vi "RemoteVI Complex Fixture Arrange.vi"(0 "Fixture":path, 1 "Views":path[](array[path]), 11 "error in":errorcluster) -> (4 "problems":string[](array[string]), 15 "error out":errorcluster)   [LabVIEW 2020]
doc: "Build tool of RemoteVI Complex Fixture.vi: run it after RemoteVI Complex Fixture Paste.vi, with the fixture idle; it can be run again (every step sets, nothing is added). Lays the panel out: each control is moved (GObject Move) into its pane (0 left, 1 toolbar, 2 main) or into a page of the tab control Settings and placed at fixed panel-area coordinates (the pane coordinates are the wanted point minus where the pane's 0,0 lands: CvtPaneToPanelCoords, CvtPanelToScreenCoords, minus Panel Bounds - placing relative to the pane's Position drifted from run to run) or relative to Settings. The toolbar holds Inspector, View, Stop and Status, the left pane Nav, Results and Steps (taller than the pane, so it scrolls) and the hidden Log Path and error out, the main pane Settings; page Acquisition holds Channel, Rate, Level and Data File, page Display holds Scope, page Viewer (added with Add Page when the tab has two) the subpanel Viewer. Then: pages named Acquisition, Display and Viewer with fixed 110 px tabs, Stop and Inspector switch when released, Data File with its browse button, Results with column headers and three rows, Steps three elements high, tip strips on Rate, on Gain inside Channel and on Nav, the main pane scaling Settings with the pane (Pane Set Scaling, Scale Single Object), the left pane's vertical scrollbar always on, the window 1180 x 760; in View A, View B and the inspector (Views) the Quit switches hidden and tip strips set. Saves the fixture and the views. problems lists every row or step that returned an error, with its code; the run goes on."
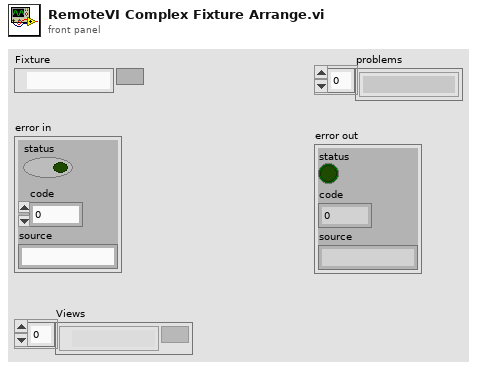
[diagram p1: front panel]
types:
  T1 = enum16{"Always On", "Always Off", "Off While Running"}
  T2 = enum16{"No Scaling", "Scale All Objects", "Scale Single Object"}
  T3 = cluster{"Left":i32, "Top":i32, "Right":i32, "Bottom":i32}
  T4 = typedef "LVRectTypeDef.ctl" = cluster{"left":i16, "top":i16, "right":i16, "bottom":i16}
  T5 = typedef "LVPositionTypeDef.ctl" = cluster{"Left":i32, "Top":i32}
  T6 = typedef "LVPointTypeDef.ctl" = cluster{"Horizontal":i16, "Vertical":i16}
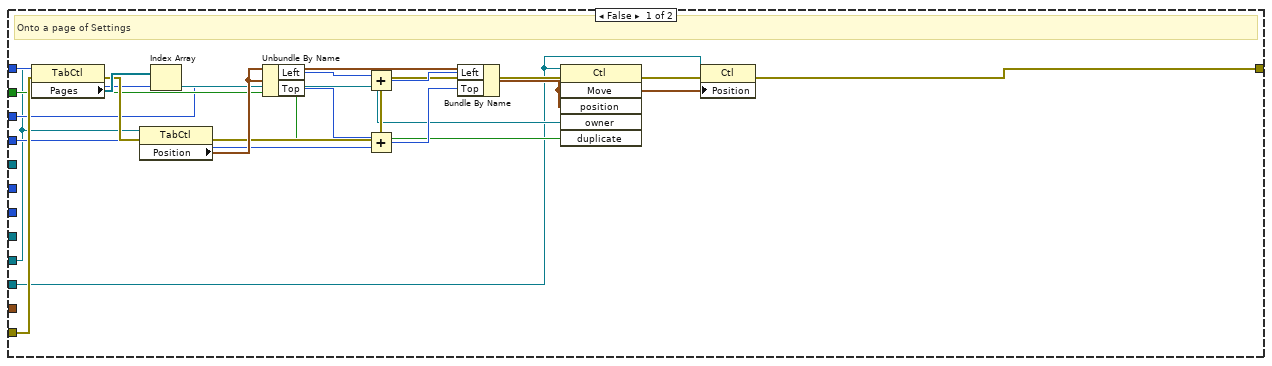
[diagram p2: hidden frame]
diagram:
  w221 = FALSE  # hidden
  w220 = string[] ["Apply view A", "Run view B", "Apply the note"]  # tips
  w219 = string[] ["A Apply", "B Run", "Apply"]  # tip labels
  w218 = string[] ["A Quit", "B Quit", "Inspector Quit"]  # quit labels
  w215 = "VertScrollbarVisibility %d"  # fmt
  w212 = T1."Always On"  # always on
  w209 = "Set Scaling %d"  # fmt
  w206 = T2."Scale Single Object"  # scale single object
  w204 = 2  # two
  w202 = "Status Label.Visible %d"  # fmt
  w198 = FALSE  # value
  w194 = string[] ["Status"]  # Status
  w192 = "View Label.Visible %d"  # fmt
  w188 = FALSE  # value
  w184 = string[] ["View"]  # View
  w182 = "Nav TipStrip %d"  # fmt
  w178 = "Pick a section"  # value
  w174 = string[] ["Nav"]  # Nav
  w172 = "Gain TipStrip %d"  # fmt
  w168 = "Channel gain"  # value
  w164 = string[] ["Gain"]  # Gain
  w162 = "Rate TipStrip %d"  # fmt
  w158 = "Sample rate"  # value
  w154 = string[] ["Rate"]  # Rate
  w152 = "Steps Number of Rows %d"  # fmt
  w148 = u32 3  # value
  w145 = refnum<vi> refnum  # class
  w141 = string[] ["Steps"]  # Steps
  w139 = "Results Value %d"  # fmt
  w135 = string[][] [["Init", "1"], ["Run", "2"], ["Stop", "3"]]  # value
  w132 = refnum<vi> refnum  # class
  w128 = string[] ["Results"]  # Results
  w126 = "Results Column Header Strings[] %d"  # fmt
  w122 = string[] ["Step", "Value"]  # value
  w119 = refnum<vi> refnum  # class
  w115 = string[] ["Results"]  # Results
  w113 = "Results Visible Items:Column Headers Visible %d"  # fmt
  w109 = TRUE  # value
  w106 = refnum<vi> refnum  # class
  w102 = string[] ["Results"]  # Results
  w100 = "Data File Browse Button:Visible %d"  # fmt
  w96 = TRUE  # value
  w93 = refnum<vi> refnum  # class
  w89 = string[] ["Data File"]  # Data File
  w87 = "error out Visible %d"  # fmt
  w83 = FALSE  # value
  w79 = string[] ["error out"]  # error out
  w77 = "Log Path Visible %d"  # fmt
  w73 = FALSE  # value
  w69 = string[] ["Log Path"]  # Log Path
  w67 = "Inspector Mechanical Action %d"  # fmt
  w63 = u32 1  # value
  w60 = refnum<vi> refnum  # class
  w56 = string[] ["Inspector"]  # Inspector
  w54 = "Stop Mechanical Action %d"  # fmt
  w50 = u32 1  # value
  w47 = refnum<vi> refnum  # class
  w43 = string[] ["Stop"]  # Stop
  w36 = FALSE  # no duplicate
  w35 = cluster{"Left":i32, "Top":i32}[] [{"Left"=300, "Top"=6}, {"Left"=420, "Top"=7}, {"Left"=14, "Top"=28}, {"Left"=120, "Top"=28}, {"Left"=14, "Top"=84}, {"Left"=14, "Top"=310}, {"Left"=14, "Top"=600}, {"Left"=14, "Top"=860}, {"Left"=14, "Top"=900}, {"Left"=300, "Top"=52}, {"Left"=20, "Top"=50}, {"Left"=230, "Top"=40}, {"Left"=390, "Top"=40}, {"Left"=20, "Top"=220}, {"Left"=10, "Top"=40}, {"Left"=20, "Top"=50}]  # offsets
  w34 = i32[] [-1, -1, -1, -1, -1, -1, -1, -1, -1, -1, 0, 0, 0, 0, 1, 2]  # pages
  w33 = i32[] [1, 1, 0, 0, 0, 0, 0, 0, 0, 2, 2, 2, 2, 2, 2, 2]  # panes
  w32 = string[] ["View", "Status", "Inspector", "Stop", "Nav", "Results", "Steps", "Log Path", "error out", "Settings", "Channel", "Rate", "Level", "Data File", "Scope", "Viewer"]  # labels
  w29 = string[] ["Acquisition", "Display", "Viewer"]  # page names
  w25 = 3  # three
  w21 = cluster{"Width":i32, "Height":i32} {"Width"=110, "Height"=23}  # tab dimension
  w20 = 2  # fixed tab size
  w17 = refnum<vi> refnum  # tab class
  w15 = 1  # one
  w14 = 0  # zero
  w11 = string[] ["Settings", "Gain"]  # settings
  w9 = T3 {"Left"=80, "Top"=80, "Right"=1260, "Bottom"=840}  # window
  # "Lay the panel out, then save"
  n1 = for {
    tunnel: "Views" -> [w229] mode=indexing
    tunnel: w218 -> [w230] mode=indexing
    tunnel: w219 -> [w231] mode=indexing
    tunnel: w220 -> [w232] mode=indexing
    tunnel: w221 -> [w233]
    tunnel: w14 -> [w234]
    tunnel: w15 -> [w235]
    tunnel: [w251] -> w222 mode=indexing
    w250 = "view %s %d"  # fmt
    # "Each view"
    n2 = Open VI Reference(vi path=w229) -> (vi reference=w236:refnum<vi>, error out=w237:errorcluster)  [unwired: 5 in]
    n3 = Build Array(w230, w231) -> (w240:string[])
    n4 = property class="VI"(reference=w236, error in=w237) -> (error out=w238:errorcluster, "Front Panel"=w239:refnum<vi>)  [unwired: 1 out]
    n5 = call "RemoteVI Complex Fixture Find Controls.vi"("Panel"=w239, "labels"=w240, "error in"=w238) -> ("Controls"=w241:refnum<vi>[], "error out"=w242:errorcluster)  [unwired: 11 in]
    n6 = Index Array(array=w241, index=w234) -> (element=w243:refnum<vi>)
    n7 = Index Array(array=w241, index=w235) -> (element=w244:refnum<vi>)
    n8 = property class="Ctl"(reference=w243, error in=w242, "Visible"=w233) -> (error out=w245:errorcluster)  [unwired: 1 out]
    n9 = property class="Ctl"(reference=w244, error in=w245, "TipStrip"=w232) -> (error out=w246:errorcluster)  [unwired: 1 out]
    n10 = invoke class="VI" method="Save.Instrument"(reference=w236, error in=w246) -> (error out=w247:errorcluster)  [unwired: 4 in, 5 out]
    n11 = Close Reference(reference=w236, error in (no error)=w247) -> (error out=w248:errorcluster)
    n12 = Unbundle By Name(w248) -> ("code"=w249:i32)
    n13 = Format Into String(format string=w250, w230, w249) -> (resulting string=w251:string)  [unwired: 2 in, 1 out]
  }
  n14 = Open VI Reference(vi path="Fixture", error in (no error)="error in") -> (vi reference=w3:refnum<vi>, error out=w4:errorcluster)  [unwired: 4 in]
  n15 = property class="VI"(reference=w3) -> ("Front Panel Window:Panel Bounds"=w37:T4)  [unwired: 1 in, 2 out]
  n16 = property class="VI"(reference=w3, error in=w4) -> (error out=w5:errorcluster, "Front Panel"=w6:refnum<vi>)  [unwired: 1 out]
  n17 = property class="Pnl"(reference=w6, error in=w5) -> (error out=w7:errorcluster, "Panes[]"=w8:refnum<vi>[])  [unwired: 1 out]
  n18 = Unbundle By Name(w37) -> ("left"=w38:i16, "top"=w39:i16)
  n19 = property class="VI"(reference=w3, error in=w7, "Front Panel Window:Panel Bounds"=w9) -> (error out=w10:errorcluster)  [unwired: 1 out]
  n20 = Index Array(array=w8, index=w204) -> (element=w205:refnum<vi>)
  n21 = Index Array(array=w8, index=w14) -> (element=w211:refnum<vi>)
  n22 = call "RemoteVI Complex Fixture Find Controls.vi"("Panel"=w6, "labels"=w11, "error in"=w10) -> ("Controls"=w12:refnum<vi>[], "error out"=w13:errorcluster)  [unwired: 11 in]
  n23 = Index Array(array=w12, index=w14) -> (element=w16:refnum<vi>)
  n24 = To More Specific Class(target class=w17, reference=w16, error in=w13) -> (specific class reference=w18:refnum<vi>, error out=w19:errorcluster)
  n25 = property class="TabCtl"(reference=w18, error in=w19, "Tab Size"=w20, "Fixed Tab Dimension"=w21) -> (error out=w22:errorcluster, "Pages"=w23:refnum<vi>[])  [unwired: 1 out]
  n26 = Array Size(array=w23) -> (size(s)=w24:i32)
  n27 = Less?(x=w24, y=w25) -> (x < y?=w26:bool)
  n28 = case shown="True" w26 {
    tunnel: w18 -> [_ w254]
    tunnel: w22 -> [w252 w255]
    tunnel: w23 -> [w253 _]
    tunnel: [w253 w260] -> w27
    tunnel: [w252 w259] -> w28
    frame False {
    }
    frame True {
      w257 = TRUE  # after
      w256 = 1  # after page 1
      # "Two pages: add the third (Viewer)"
      n29 = invoke class="TabCtl" method="Add Page"(reference=w254, error in=w255, "Page"=w256, "After"=w257) -> (error out=w258:errorcluster)  [unwired: 1 in, 4 out]
      n30 = property class="TabCtl"(reference=w254, error in=w258) -> (error out=w259:errorcluster, "Pages"=w260:refnum<vi>[])  [unwired: 1 out]
    }
  }
  n31 = for {
    tunnel: w29 -> [w262] mode=indexing
    tunnel: w27 -> [w261] mode=indexing
    shift-right: [w264] -> w30
    shift-left: w28 -> [w263]
    # "Name the pages"
    n32 = property class="Page"(reference=w261, error in=w263, "Page Label"=w262, "TabCaption"=w262) -> (error out=w264:errorcluster)  [unwired: 1 out]
  }
  n33 = call <vilib>:"Clear Errors.vi"("error in (no error)"=w30) -> ("error out"=w31:errorcluster)  [unwired: 5 in, 1 out]
  n34 = for {
    tunnel: w32 -> [w265] mode=indexing
    tunnel: w33 -> [w266] mode=indexing
    tunnel: w34 -> [w267] mode=indexing
    tunnel: w35 -> [w268] mode=indexing
    tunnel: w36 -> [w272]
    tunnel: w6 -> [w269]
    tunnel: w8 -> [w270]
    tunnel: w38 -> [w274]
    tunnel: w39 -> [w275]
    tunnel: w18 -> [w271]
    tunnel: w31 -> [w273]
    tunnel: [w287] -> w41
    tunnel: [w290] -> w40 mode=indexing
    w289 = "%s %d"  # fmt
    w279 = 0  # zero
    # "Move each control into its pane or page and place it"
    n35 = Build Array(w265) -> (w276:string[])
    n36 = Less Than 0?(x=w267) -> (x < 0?=w284:bool)
    n37 = Unbundle By Name(w268) -> ("Left"=w285:i32, "Top"=w286:i32)
    n38 = Index Array(array=w270, index=w266) -> (element=w281:refnum<vi>)
    n39 = call "RemoteVI Complex Fixture Find Controls.vi"("Panel"=w269, "labels"=w276, "error in"=w273) -> ("Controls"=w277:refnum<vi>[], "error out"=w278:errorcluster)  [unwired: 11 in]
    n40 = property class="Pane"(reference=w281, error in=w278) -> (error out=w282:errorcluster, "Position"=w283:T5)  [unwired: 1 out]
    n41 = Index Array(array=w277, index=w279) -> (element=w280:refnum<vi>)
    n42 = case shown="True" w284 {
      tunnel: w267 -> [w293 _]
      tunnel: w272 -> [w296 w314]
      tunnel: w285 -> [w294 w312]
      tunnel: w286 -> [w295 w313]
      tunnel: w269 -> [_ w316]
      tunnel: w274 -> [_ w317]
      tunnel: w275 -> [_ w318]
      tunnel: w281 -> [_ w311]
      tunnel: w271 -> [w292 _]
      tunnel: w280 -> [w291 w310]
      tunnel: w283 -> [_ _]
      tunnel: w282 -> [w297 w315]
      tunnel: [w309 w333] -> w287
      frame False {
        # "Onto a page of Settings"
        n43 = property class="TabCtl"(reference=w292, error in=w297) -> (error out=w298:errorcluster, "Pages"=w299:refnum<vi>[])  [unwired: 1 out]
        n44 = property class="TabCtl"(reference=w292, error in=w298) -> (error out=w301:errorcluster, "Position"=w302:T5)  [unwired: 1 out]
        n45 = Index Array(array=w299, index=w293) -> (element=w300:refnum<vi>)
        n46 = Unbundle By Name(w302) -> ("Left"=w303:i32, "Top"=w304:i32)
        n47 = Add(x=w303, y=w294) -> (x+y=w305:i32)
        n48 = Add(x=w304, y=w295) -> (x+y=w306:i32)
        n49 = Bundle By Name(cluster=w302, "Left"=w305, "Top"=w306) -> (w307:T5)
        n50 = invoke class="Ctl" method="Move"(reference=w291, error in=w301, "position"=w307, "owner"=w300, "duplicate"=w296) -> (error out=w308:errorcluster)  [unwired: 1 in, 5 out]
        n51 = property class="Ctl"(reference=w291, error in=w308, "Position"=w307) -> (error out=w309:errorcluster)  [unwired: 1 out]
      }
      frame True {
        w330 = cluster{"Left":i32, "Top":i32} {"Left"=0, "Top"=0}  # position
        w319 = cluster{"Horizontal":i32, "Vertical":i32} {"Horizontal"=0, "Vertical"=0}  # pane origin
        # "Into the pane"
        n52 = invoke class="Pane" method="CvtPaneToPanelCoords"(reference=w311, error in=w315, "PaneCoords"=w319) -> (error out=w320:errorcluster, "PanelCoords"=w321:T6)  [unwired: 2 in, 3 out]
        n53 = invoke class="Pnl" method="CvtPanelToScreenCoords"(reference=w316, error in=w320, "PanelCoords"=w321) -> (error out=w322:errorcluster, "ScreenCoords"=w323:T6)  [unwired: 2 in, 3 out]
        n54 = Unbundle By Name(w323) -> ("Horizontal"=w324:i16, "Vertical"=w325:i16)
        n55 = Subtract(x=w324, y=w317) -> (x-y=w326:i16)
        n56 = Subtract(x=w325, y=w318) -> (x-y=w327:i16)
        n57 = Subtract(x=w312, y=w326) -> (x-y=w328:i32)
        n58 = Subtract(x=w313, y=w327) -> (x-y=w329:i32)
        n59 = Bundle By Name(cluster=w330, "Left"=w328, "Top"=w329) -> (w331:cluster{"Left":i32, "Top":i32})
        n60 = invoke class="Ctl" method="Move"(reference=w310, error in=w322, "position"=w331, "owner"=w311, "duplicate"=w314) -> (error out=w332:errorcluster)  [unwired: 1 in, 5 out]
        n61 = property class="Ctl"(reference=w310, error in=w332, "Position"=w331) -> (error out=w333:errorcluster)  [unwired: 1 out]
      }
    }
    n62 = Unbundle By Name(w287) -> ("code"=w288:i32)
    n63 = Format Into String(format string=w289, w265, w288) -> (resulting string=w290:string)  [unwired: 2 in, 1 out]
  }
  n64 = call <vilib>:"Clear Errors.vi"("error in (no error)"=w41) -> ("error out"=w42:errorcluster)  [unwired: 5 in, 1 out]
  n65 = call "RemoteVI Complex Fixture Find Controls.vi"("Panel"=w6, "labels"=w43, "error in"=w42) -> ("Controls"=w44:refnum<vi>[], "error out"=w45:errorcluster)  [unwired: 11 in]
  n66 = Index Array(array=w44, index=w14) -> (element=w46:refnum<vi>)
  n67 = To More Specific Class(target class=w47, reference=w46, error in=w45) -> (specific class reference=w48:refnum<vi>, error out=w49:errorcluster)
  n68 = property class="Bool"(reference=w48, error in=w49, "Mechanical Action"=w50) -> (error out=w51:errorcluster)  [unwired: 1 out]
  n69 = Unbundle By Name(w51) -> ("code"=w52:i32)
  n70 = call <vilib>:"Clear Errors.vi"("error in (no error)"=w51) -> ("error out"=w53:errorcluster)  [unwired: 5 in, 1 out]
  n71 = Format Into String(format string=w54, w52) -> (resulting string=w55:string)  [unwired: 2 in, 1 out]
  n72 = call "RemoteVI Complex Fixture Find Controls.vi"("Panel"=w6, "labels"=w56, "error in"=w53) -> ("Controls"=w57:refnum<vi>[], "error out"=w58:errorcluster)  [unwired: 11 in]
  n73 = Index Array(array=w57, index=w14) -> (element=w59:refnum<vi>)
  n74 = To More Specific Class(target class=w60, reference=w59, error in=w58) -> (specific class reference=w61:refnum<vi>, error out=w62:errorcluster)
  n75 = property class="Bool"(reference=w61, error in=w62, "Mechanical Action"=w63) -> (error out=w64:errorcluster)  [unwired: 1 out]
  n76 = Unbundle By Name(w64) -> ("code"=w65:i32)
  n77 = call <vilib>:"Clear Errors.vi"("error in (no error)"=w64) -> ("error out"=w66:errorcluster)  [unwired: 5 in, 1 out]
  n78 = Format Into String(format string=w67, w65) -> (resulting string=w68:string)  [unwired: 2 in, 1 out]
  n79 = call "RemoteVI Complex Fixture Find Controls.vi"("Panel"=w6, "labels"=w69, "error in"=w66) -> ("Controls"=w70:refnum<vi>[], "error out"=w71:errorcluster)  [unwired: 11 in]
  n80 = Index Array(array=w70, index=w14) -> (element=w72:refnum<vi>)
  n81 = property class="Ctl"(reference=w72, error in=w71, "Visible"=w73) -> (error out=w74:errorcluster)  [unwired: 1 out]
  n82 = Unbundle By Name(w74) -> ("code"=w75:i32)
  n83 = call <vilib>:"Clear Errors.vi"("error in (no error)"=w74) -> ("error out"=w76:errorcluster)  [unwired: 5 in, 1 out]
  n84 = Format Into String(format string=w77, w75) -> (resulting string=w78:string)  [unwired: 2 in, 1 out]
  n85 = call "RemoteVI Complex Fixture Find Controls.vi"("Panel"=w6, "labels"=w79, "error in"=w76) -> ("Controls"=w80:refnum<vi>[], "error out"=w81:errorcluster)  [unwired: 11 in]
  n86 = Index Array(array=w80, index=w14) -> (element=w82:refnum<vi>)
  n87 = property class="Ctl"(reference=w82, error in=w81, "Visible"=w83) -> (error out=w84:errorcluster)  [unwired: 1 out]
  n88 = Unbundle By Name(w84) -> ("code"=w85:i32)
  n89 = call <vilib>:"Clear Errors.vi"("error in (no error)"=w84) -> ("error out"=w86:errorcluster)  [unwired: 5 in, 1 out]
  n90 = Format Into String(format string=w87, w85) -> (resulting string=w88:string)  [unwired: 2 in, 1 out]
  n91 = call "RemoteVI Complex Fixture Find Controls.vi"("Panel"=w6, "labels"=w89, "error in"=w86) -> ("Controls"=w90:refnum<vi>[], "error out"=w91:errorcluster)  [unwired: 11 in]
  n92 = Index Array(array=w90, index=w14) -> (element=w92:refnum<vi>)
  n93 = To More Specific Class(target class=w93, reference=w92, error in=w91) -> (specific class reference=w94:refnum<vi>, error out=w95:errorcluster)
  n94 = property class="Path"(reference=w94, error in=w95, "Browse Button:Visible"=w96) -> (error out=w97:errorcluster)  [unwired: 1 out]
  n95 = Unbundle By Name(w97) -> ("code"=w98:i32)
  n96 = call <vilib>:"Clear Errors.vi"("error in (no error)"=w97) -> ("error out"=w99:errorcluster)  [unwired: 5 in, 1 out]
  n97 = Format Into String(format string=w100, w98) -> (resulting string=w101:string)  [unwired: 2 in, 1 out]
  n98 = call "RemoteVI Complex Fixture Find Controls.vi"("Panel"=w6, "labels"=w102, "error in"=w99) -> ("Controls"=w103:refnum<vi>[], "error out"=w104:errorcluster)  [unwired: 11 in]
  n99 = Index Array(array=w103, index=w14) -> (element=w105:refnum<vi>)
  n100 = To More Specific Class(target class=w106, reference=w105, error in=w104) -> (specific class reference=w107:refnum<vi>, error out=w108:errorcluster)
  n101 = property class="Tbl"(reference=w107, error in=w108, "Visible Items:Column Headers Visible"=w109) -> (error out=w110:errorcluster)  [unwired: 1 out]
  n102 = Unbundle By Name(w110) -> ("code"=w111:i32)
  n103 = call <vilib>:"Clear Errors.vi"("error in (no error)"=w110) -> ("error out"=w112:errorcluster)  [unwired: 5 in, 1 out]
  n104 = Format Into String(format string=w113, w111) -> (resulting string=w114:string)  [unwired: 2 in, 1 out]
  n105 = call "RemoteVI Complex Fixture Find Controls.vi"("Panel"=w6, "labels"=w115, "error in"=w112) -> ("Controls"=w116:refnum<vi>[], "error out"=w117:errorcluster)  [unwired: 11 in]
  n106 = Index Array(array=w116, index=w14) -> (element=w118:refnum<vi>)
  n107 = To More Specific Class(target class=w119, reference=w118, error in=w117) -> (specific class reference=w120:refnum<vi>, error out=w121:errorcluster)
  n108 = property class="Tbl"(reference=w120, error in=w121, "Column Header Strings[]"=w122) -> (error out=w123:errorcluster)  [unwired: 1 out]
  n109 = Unbundle By Name(w123) -> ("code"=w124:i32)
  n110 = call <vilib>:"Clear Errors.vi"("error in (no error)"=w123) -> ("error out"=w125:errorcluster)  [unwired: 5 in, 1 out]
  n111 = Format Into String(format string=w126, w124) -> (resulting string=w127:string)  [unwired: 2 in, 1 out]
  n112 = call "RemoteVI Complex Fixture Find Controls.vi"("Panel"=w6, "labels"=w128, "error in"=w125) -> ("Controls"=w129:refnum<vi>[], "error out"=w130:errorcluster)  [unwired: 11 in]
  n113 = Index Array(array=w129, index=w14) -> (element=w131:refnum<vi>)
  n114 = To More Specific Class(target class=w132, reference=w131, error in=w130) -> (specific class reference=w133:refnum<vi>, error out=w134:errorcluster)
  n115 = property class="Tbl"(reference=w133, error in=w134, "Value"=w135) -> (error out=w136:errorcluster)  [unwired: 1 out]
  n116 = Unbundle By Name(w136) -> ("code"=w137:i32)
  n117 = call <vilib>:"Clear Errors.vi"("error in (no error)"=w136) -> ("error out"=w138:errorcluster)  [unwired: 5 in, 1 out]
  n118 = Format Into String(format string=w139, w137) -> (resulting string=w140:string)  [unwired: 2 in, 1 out]
  n119 = call "RemoteVI Complex Fixture Find Controls.vi"("Panel"=w6, "labels"=w141, "error in"=w138) -> ("Controls"=w142:refnum<vi>[], "error out"=w143:errorcluster)  [unwired: 11 in]
  n120 = Index Array(array=w142, index=w14) -> (element=w144:refnum<vi>)
  n121 = To More Specific Class(target class=w145, reference=w144, error in=w143) -> (specific class reference=w146:refnum<vi>, error out=w147:errorcluster)
  n122 = property class="Arr"(reference=w146, error in=w147, "Number of Rows"=w148) -> (error out=w149:errorcluster)  [unwired: 1 out]
  n123 = Unbundle By Name(w149) -> ("code"=w150:i32)
  n124 = call <vilib>:"Clear Errors.vi"("error in (no error)"=w149) -> ("error out"=w151:errorcluster)  [unwired: 5 in, 1 out]
  n125 = Format Into String(format string=w152, w150) -> (resulting string=w153:string)  [unwired: 2 in, 1 out]
  n126 = call "RemoteVI Complex Fixture Find Controls.vi"("Panel"=w6, "labels"=w154, "error in"=w151) -> ("Controls"=w155:refnum<vi>[], "error out"=w156:errorcluster)  [unwired: 11 in]
  n127 = Index Array(array=w155, index=w14) -> (element=w157:refnum<vi>)
  n128 = property class="Ctl"(reference=w157, error in=w156, "TipStrip"=w158) -> (error out=w159:errorcluster)  [unwired: 1 out]
  n129 = Unbundle By Name(w159) -> ("code"=w160:i32)
  n130 = call <vilib>:"Clear Errors.vi"("error in (no error)"=w159) -> ("error out"=w161:errorcluster)  [unwired: 5 in, 1 out]
  n131 = Format Into String(format string=w162, w160) -> (resulting string=w163:string)  [unwired: 2 in, 1 out]
  n132 = call "RemoteVI Complex Fixture Find Controls.vi"("Panel"=w6, "labels"=w164, "error in"=w161) -> ("Controls"=w165:refnum<vi>[], "error out"=w166:errorcluster)  [unwired: 11 in]
  n133 = Index Array(array=w165, index=w14) -> (element=w167:refnum<vi>)
  n134 = property class="Ctl"(reference=w167, error in=w166, "TipStrip"=w168) -> (error out=w169:errorcluster)  [unwired: 1 out]
  n135 = Unbundle By Name(w169) -> ("code"=w170:i32)
  n136 = call <vilib>:"Clear Errors.vi"("error in (no error)"=w169) -> ("error out"=w171:errorcluster)  [unwired: 5 in, 1 out]
  n137 = Format Into String(format string=w172, w170) -> (resulting string=w173:string)  [unwired: 2 in, 1 out]
  n138 = call "RemoteVI Complex Fixture Find Controls.vi"("Panel"=w6, "labels"=w174, "error in"=w171) -> ("Controls"=w175:refnum<vi>[], "error out"=w176:errorcluster)  [unwired: 11 in]
  n139 = Index Array(array=w175, index=w14) -> (element=w177:refnum<vi>)
  n140 = property class="Ctl"(reference=w177, error in=w176, "TipStrip"=w178) -> (error out=w179:errorcluster)  [unwired: 1 out]
  n141 = Unbundle By Name(w179) -> ("code"=w180:i32)
  n142 = call <vilib>:"Clear Errors.vi"("error in (no error)"=w179) -> ("error out"=w181:errorcluster)  [unwired: 5 in, 1 out]
  n143 = Format Into String(format string=w182, w180) -> (resulting string=w183:string)  [unwired: 2 in, 1 out]
  n144 = call "RemoteVI Complex Fixture Find Controls.vi"("Panel"=w6, "labels"=w184, "error in"=w181) -> ("Controls"=w185:refnum<vi>[], "error out"=w186:errorcluster)  [unwired: 11 in]
  n145 = Index Array(array=w185, index=w14) -> (element=w187:refnum<vi>)
  n146 = property class="Ctl"(reference=w187, error in=w186, "Label.Visible"=w188) -> (error out=w189:errorcluster)  [unwired: 1 out]
  n147 = Unbundle By Name(w189) -> ("code"=w190:i32)
  n148 = call <vilib>:"Clear Errors.vi"("error in (no error)"=w189) -> ("error out"=w191:errorcluster)  [unwired: 5 in, 1 out]
  n149 = Format Into String(format string=w192, w190) -> (resulting string=w193:string)  [unwired: 2 in, 1 out]
  n150 = call "RemoteVI Complex Fixture Find Controls.vi"("Panel"=w6, "labels"=w194, "error in"=w191) -> ("Controls"=w195:refnum<vi>[], "error out"=w196:errorcluster)  [unwired: 11 in]
  n151 = Index Array(array=w195, index=w14) -> (element=w197:refnum<vi>)
  n152 = property class="Ctl"(reference=w197, error in=w196, "Label.Visible"=w198) -> (error out=w199:errorcluster)  [unwired: 1 out]
  n153 = Unbundle By Name(w199) -> ("code"=w200:i32)
  n154 = call <vilib>:"Clear Errors.vi"("error in (no error)"=w199) -> ("error out"=w201:errorcluster)  [unwired: 5 in, 1 out]
  n155 = Format Into String(format string=w202, w200) -> (resulting string=w203:string)  [unwired: 2 in, 1 out]
  n156 = invoke class="Pane" method="Set Scaling"(reference=w205, error in=w201, "ScalingMode"=w206, "ScalableObj"=w16) -> (error out=w207:errorcluster)  [unwired: 1 in, 4 out]
  n157 = property class="Pane"(reference=w211, error in=w207, "VertScrollbarVisibility"=w212) -> (error out=w213:errorcluster)  [unwired: 1 out]
  n158 = Unbundle By Name(w207) -> ("code"=w208:i32)
  n159 = Format Into String(format string=w209, w208) -> (resulting string=w210:string)  [unwired: 2 in, 1 out]
  n160 = Unbundle By Name(w213) -> ("code"=w214:i32)
  n161 = Merge Errors(w199, w213) -> (w224:errorcluster)
  n162 = Format Into String(format string=w215, w214) -> (resulting string=w216:string)  [unwired: 2 in, 1 out]
  n163 = call <vilib>:"Clear Errors.vi"("error in (no error)"=w224) -> ("error out"=w225:errorcluster)  [unwired: 5 in, 1 out]
  n164 = Build Array (concatenate)(w40, w55, w68, w78, w88, w101, w114, w127, w140, w153, w163, w173, w183, w193, w203, w210, w216, w222) -> (→"problems":string[])
  n165 = invoke class="VI" method="Save.Instrument"(reference=w3, error in=w225) -> (reference out=w226:refnum<vi>, error out=w227:errorcluster)  [unwired: 4 in, 4 out]
  n166 = Close Reference(reference=w226, error in (no error)=w227) -> (error out=→"error out":errorcluster)
